vi "destroyMsgParser.vi"(7 "path in":path=path "C:/dev/Hexagon-VTD-Custom-Device/Libraries/VC.dll", 8 "error in (no error)":errorcluster, 11 "parserHandle":u64) -> (0 "error out":errorcluster)   [LabVIEW 2023, in "RDB.lvlib"]
uses:
  RDB.lvlib
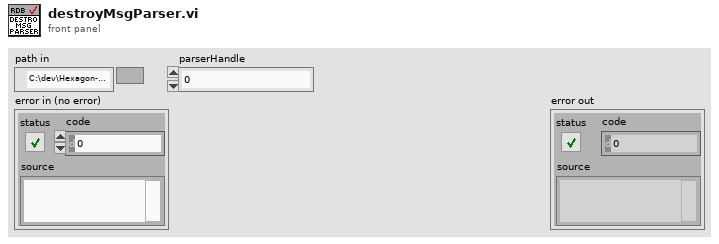
[diagram p1: front panel]
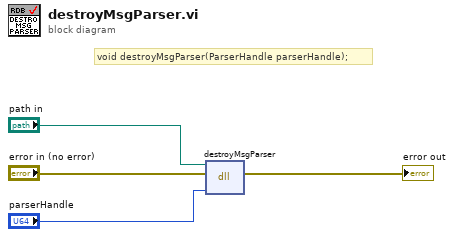
[diagram p0: block diagram]
diagram:
  # "void destroyMsgParser(ParserHandle parserHandle);"
  n1 = dll-call lib="C:/dev/Hexagon-VTD-Custom-Device/Libraries/VC.dll" fn="destroyMsgParser"(path in="path in", error in="error in (no error)", "paeseHandle"="parserHandle") -> (error out=→"error out":errorcluster)  [unwired: 3 in, 1 out]
